vi "Test WS Local Echo Server.vi"(8 "error in (no error)":errorcluster, 11 "TestCase in":refnum<class "Test Legacy Server.lvclass">) -> (0 "error out":errorcluster, 3 "TestCase out":refnum<class "Test Legacy Server.lvclass">)   [LabVIEW 2013, in "Test Legacy Server.lvclass"]
uses:
  Test Legacy Server.lvclass
  <vilib>/addons/_JKI Toolkits/VI Tester/TestCase.llb/TestCase.lvclass
  WebSockets/WebSockets.lvlib
panel:
  out "Return Headers Out":variant
  out "Return Headers":variant
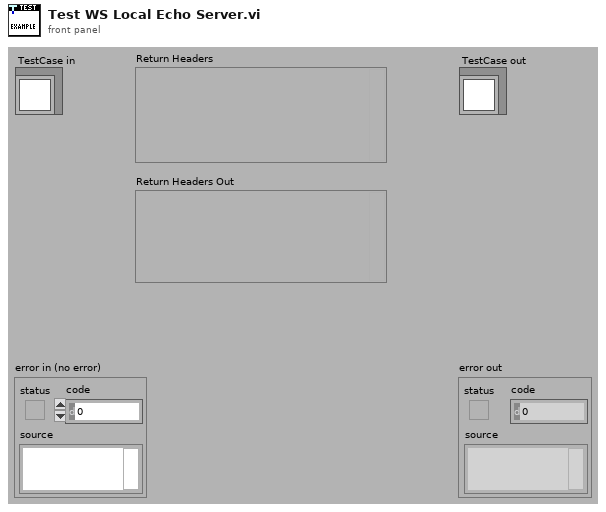
[diagram p1: front panel]
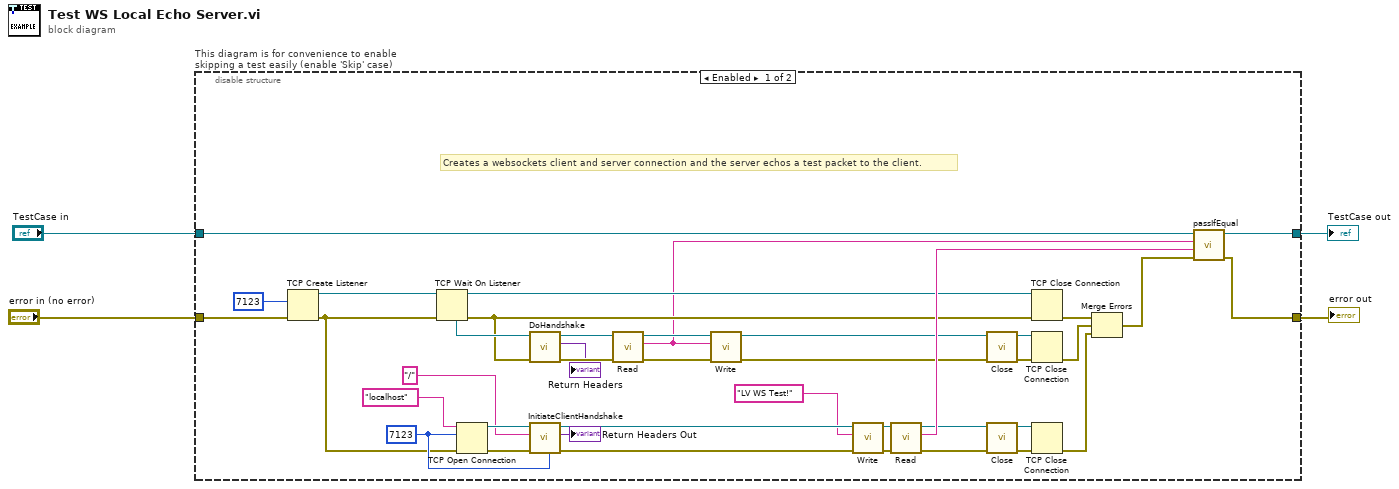
[diagram p0: block diagram]
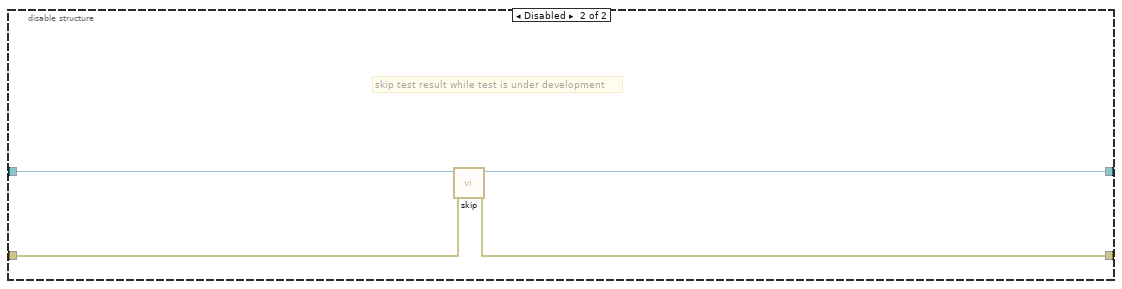
[diagram p2: hidden frame]
diagram:
  n1 = disable-structure "This diagram is for convenience to enable skipping a test easily (enable 'Skip' case)" shown="Enabled" {
    disable-tunnel: "TestCase in" -> [w35 w48]
    disable-tunnel: [w34 w46] -> w1
    disable-tunnel: [w33 w47] -> w3
    disable-tunnel: "error in (no error)" -> [w31 w45]
    frame Enabled {
      w38 = u16 7123 ("remote port or service name")
      # "Creates a websockets client and server connection and the server echos a test packet to the client."
      n2 = TCP Create Listener(8:w31, 10:u16 7123 ("port")) -> (0:w24:errorcluster, 3:w23:refnum<k5>)  [unwired: 3 in, 1 out]
      n3 = TCP Wait On Listener(8:w24, 11:w23) -> (0:w18:errorcluster, 3:w19:refnum<k5>, 4:w22:refnum<k5>)  [unwired: 2 in, 2 out]
      n4 = TCP Open Connection(address="localhost", remote port or service name=w38, error in (no error)=w24) -> (connection ID=w44:refnum<k5>, error out=w43:errorcluster)  [unwired: 2 in]
      n5 = call "DoHandshake.vi"("error in (no error)"=w18, "TCP Connection in"=w22) -> ("error out"=w30:errorcluster, "Client Headers"=→"Return Headers":variant, "WebSocket Server out"=w27:refnum<class "WebSocket Server.lvclass">)  [unwired: 6 in, 1 out]
      n6 = call "InitiateClientHandshake.vi"("remote port or service name"=w38, "error in (no error)"=w43, "request URI ('/')"="/", "TCP Connection in"=w44) -> ("error out"=w42:errorcluster, "Server Headers Out"=→"Return Headers Out":variant, "WebSocket Client out"=w41:refnum<class "WebSocket Client.lvclass">)  [unwired: 5 in]
      n7 = call "Read.vi"("error in (no error)"=w30, "WebSocket in"=w27) -> ("error out"=w29:errorcluster, "Data"=w7:string, "WebSocket out"=w28:refnum<class "WebSocket Server.lvclass">)  [unwired: 5 in, 2 out]
      n8 = call "Write.vi"("error in (no error)"=w29, "Data"=w7, "WebSocket in"=w28) -> ("error out"=w21:errorcluster, "WebSocket out"=w20:refnum<class "WebSocket Server.lvclass">)  [unwired: 7 in]
      n9 = call "Write.vi"("error in (no error)"=w42, "Data"="LV WS Test!", "WebSocket in"=w41) -> ("error out"=w40:errorcluster, "WebSocket out"=w39:refnum<class "WebSocket Client.lvclass">)  [unwired: 7 in]
      n10 = call "Read.vi"("error in (no error)"=w40, "WebSocket in"=w39) -> ("error out"=w16:errorcluster, "Data"=w26:string, "WebSocket out"=w15:refnum<class "WebSocket Client.lvclass">)  [unwired: 5 in, 2 out]
      n11 = call "Close.vi"("error in (no error)"=w21, "WebSocket in"=w20) -> ("error out"=w17:errorcluster, "TCP Connection out"=w12:refnum<k5>)  [unwired: 8 in]
      n12 = call "Close.vi"("error in (no error)"=w16, "WebSocket in"=w15) -> ("error out"=w13:errorcluster, "TCP Connection out"=w14:refnum<k5>)  [unwired: 8 in]
      n13 = TCP Close Connection(connection ID=w19, error in (no error)=w18) -> (error out=w11:errorcluster)  [unwired: 1 in, 1 out]
      n14 = TCP Close Connection(connection ID=w12, error in (no error)=w17) -> (error out=w10:errorcluster)  [unwired: 1 in, 1 out]
      n15 = TCP Close Connection(connection ID=w14, error in (no error)=w13) -> (error out=w9:errorcluster)  [unwired: 1 in, 1 out]
      n16 = Merge Errors(w11, w10, w9) -> (w8:errorcluster)
      n17 = call-dynamic "passIfEqual.vi"("error in (no error)"=w8, "y"=w26, "x"=w7, "TestCase in"=w35) -> ("error out"=w33:errorcluster, "TestCase out"=w34:refnum<class "Test Legacy Server.lvclass">)  [unwired: 6 in]
    }
    frame Disabled {
      # "skip test result while test is under development"
      n18 = call <vilib>:"skip.vi"("error in (no error)"=w45, "TestCase in"=w48) -> ("error out"=w47:errorcluster, "TestCase out"=w46:refnum<class "Test Legacy Server.lvclass">)  [unwired: 8 in]
    }
  }
  "error out" <- w3
  "TestCase out" <- w1
